vi "Demo_BjusticeData.vi"() -> ()   [LabVIEW 2021, in "RocketPlotDemo.lvlib"]
uses:
  Demo/RocketPlotDemo.lvlib
  TypeDefs/plot load data V2.ctl
  TypeDefs/plot properties V2.ctl
  TypeDefs/plot attributes V2.ctl
  TypeDefs/Plot scale axis properties.ctl
  TypeDefs/Plot general properties.ctl
  Classes/RocketPlotHandle/SubVIs/Init Options.ctl
  TypeDefs/TimeZone.ctl
  Classes/RocketPlotPanel/RocketPlotPanel.lvclass/RocketPlotPanel.ctl
  Classes/RocketPlotPanel/Read RocketPlotHandle.vi
  Classes/BjusticePlotHandle/BjusticePlotHandle.lvclass
  C:/Users/bjustice/Documents/GitHub/BluePlot/Source/Classes/RocketPlotHandle/RocketPlotHandle.lvclass
  Classes/RocketPlotPanel/RocketPlotPanel.lvclass
  C:/Program Files/National Instruments/LabVIEW 2021/vi.lib/IlluminatedG/IG OOPanel/OOPanel/Panel/Panel.lvclass
  Classes/RocketPlotHandle/Load PlotConfig.vi
  Classes/RocketPlotHandle/RocketPlotHandle.lvclass
  Classes/RocketPlotHandle/Get PlotConfig.vi
  RocketPlot.lvlib
  <userlib>/bjustice/Ring Buffer for Time Series Data Strict Accessor/Ring Buffer Strict Accessor.lvlib
  <vilib>/IlluminatedG/IG OOPanel/OOPanel/Manager/Manager.lvclass
  C:/Users/bjustice/Documents/GitHub/BluePlot/Source/Classes/BjusticePlotHandle/BjusticePlotHandle.lvclass
  C:/Users/bjustice/Documents/GitHub/BluePlot/Source/Classes/RocketPlotPanel/RocketPlotPanel.lvclass
panel:
  in  "load config":bool
  in  "get config":bool
  out "time to plot":dbl
  out "Subscribed names":i32(listbox)
  in  "Plot config":T1={"plots"=[], "X-axis"={"Name Label.Text"="", "Style"=0, "Tick Colors:Minor Tick Color"=0, "Tick Colors:Tick Color"=0, "Marker Colors:Text Color"=0, "Grid Colors:Major Color"=0, "Grid Colors:Minor Color"=0, "Mapping Mode"=0, "Flipped"=FALSE, "Name Label.Visible"=FALSE, "Name Label.Text Colors:Text Color"=0, "Scale Fit"=0, "Range:Maximum"=0.0, "Range:Minimum"=0.0, "Offset and Multiplier:Multiplier"=0.0, "Offset and Multiplier:Offset"=0.0, "Name Label.Font:Size"=0, "Marker.Font:Size"=0, "Uniform Marker Spacing?"=TRUE, "Format String"=""}, "Y-axes"=[], "General"={"Title"="", "Time to Plot"=1800.0, "Title.Visible"=FALSE, "Sidebar.Visible"=FALSE, "Plot Area:Colors:BG Color"=0, "X Scale.Plot Name"="", "X Scale.Use Plot Name"=FALSE}} {"General"."Time to Plot" format="%<%M:%S>t"}
  # "Documentation and user guide:"
  # "https://github.com/justiceb/BluePlot/blob/main/README.md"
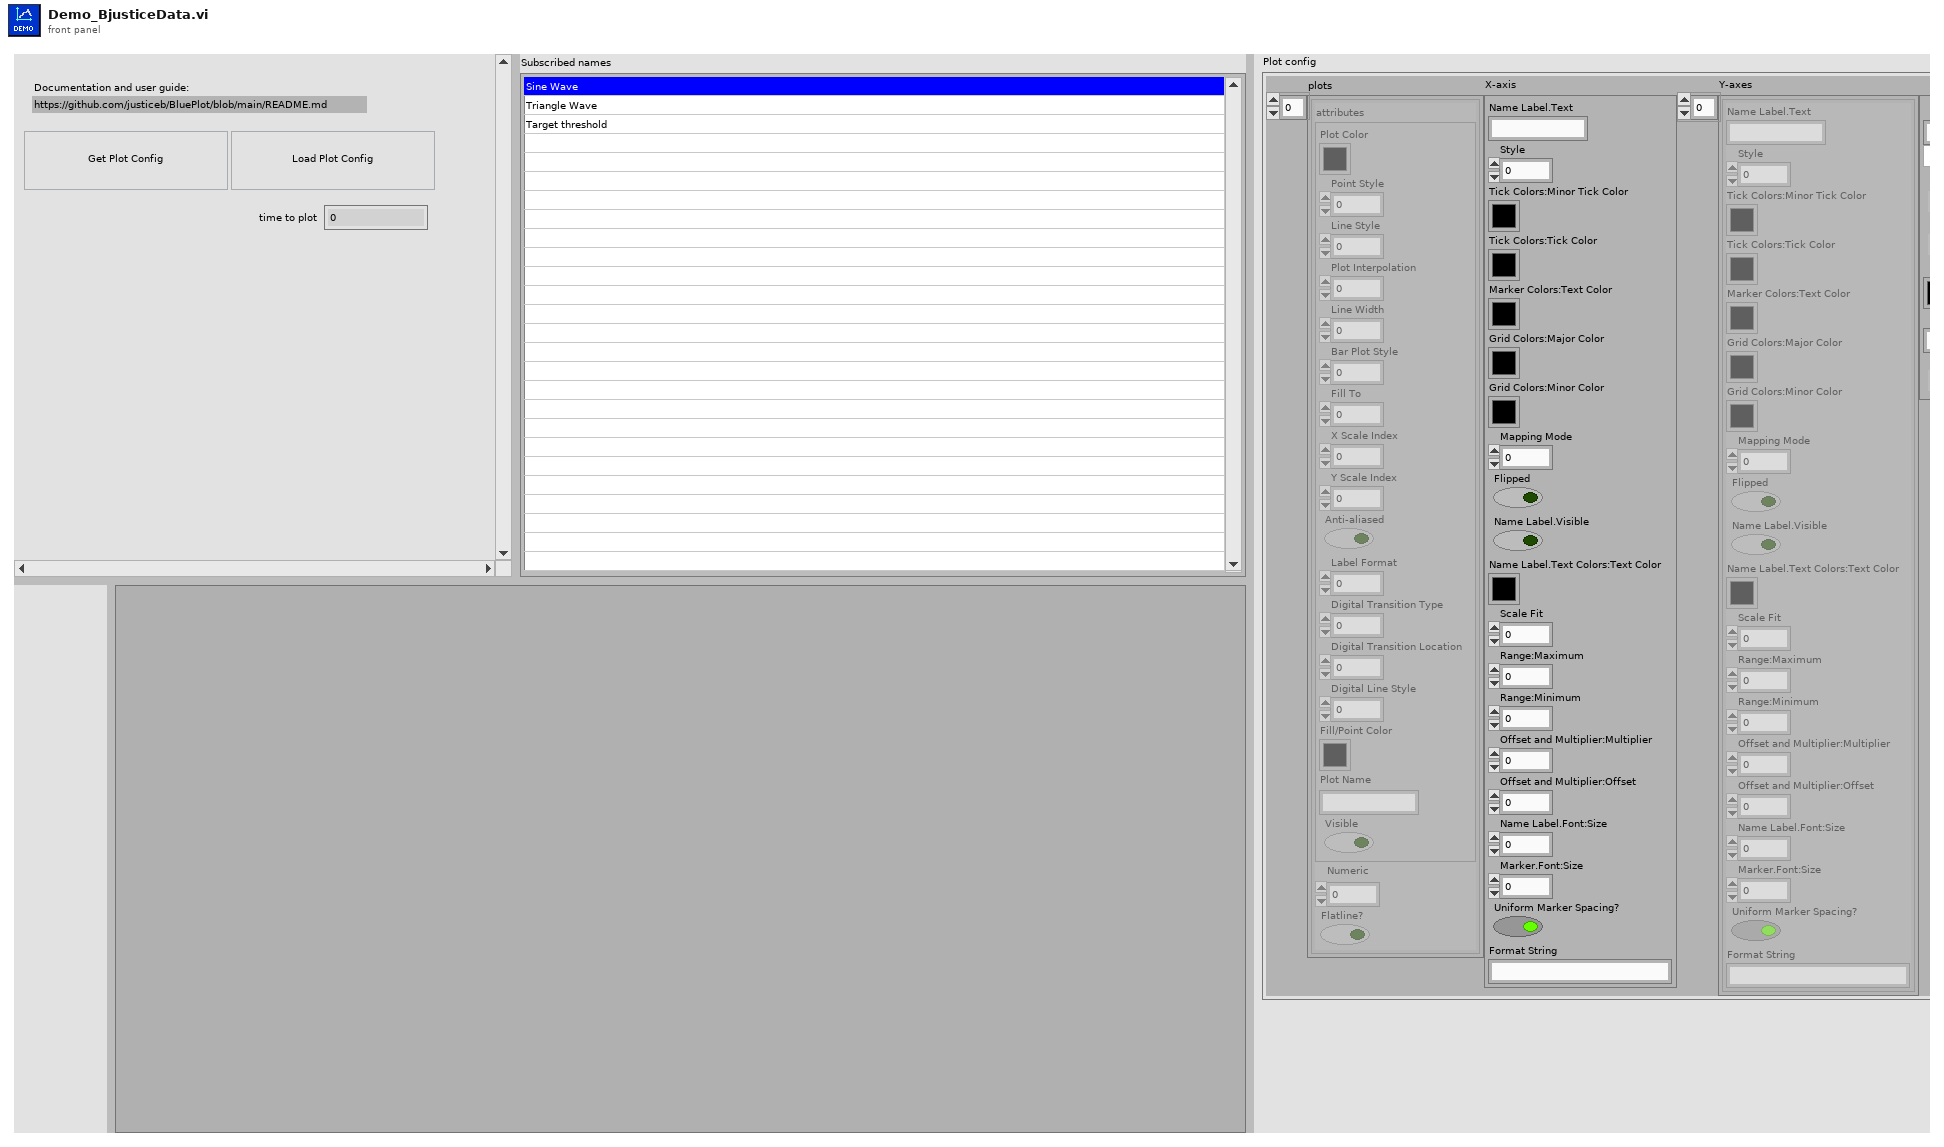
[diagram p1: front panel]
types:
  T1 = typedef "RocketPlot.lvlib/plot load data V2.ctl" = cluster{"plots":T2[], "X-axis":T4, "Y-axes":T4[], "General":T5}
  T2 = typedef "RocketPlot.lvlib/plot properties V2.ctl" = cluster{"attributes":T3, "Numeric":dbl, "Flatline?":bool}
  T3 = typedef "RocketPlot.lvlib/plot attributes V2.ctl" = cluster{"Plot Color":u32, "Point Style":u8, "Line Style":u8, "Plot Interpolation":u8, "Line Width":u8, "Bar Plot Style":u8, "Fill To":i16, "X Scale Index":u32, "Y Scale Index":u32, "Anti-aliased":bool, "Label Format":u8, "Digital Transition Type":u8, "Digital Transition Location":u8, "Digital Line Style":u8, "Fill/Point Color":u32, "Plot Name":string, "Visible":bool}
  T4 = typedef "RocketPlot.lvlib/Plot scale axis properties.ctl" = cluster{"Name Label.Text":string, "Style":u8, "Tick Colors:Minor Tick Color":u32, "Tick Colors:Tick Color":u32, "Marker Colors:Text Color":u32, "Grid Colors:Major Color":u32, "Grid Colors:Minor Color":u32, "Mapping Mode":u8, "Flipped":bool, "Name Label.Visible":bool, "Name Label.Text Colors:Text Color":u32, "Scale Fit":u8, "Range:Maximum":dbl, "Range:Minimum":dbl, "Offset and Multiplier:Multiplier":dbl, "Offset and Multiplier:Offset":dbl, "Name Label.Font:Size":u32, "Marker.Font:Size":u32, "Uniform Marker Spacing?":bool, "Format String":string}
  T5 = typedef "RocketPlot.lvlib/Plot general properties.ctl" = cluster{"Title":string, "Time to Plot":dbl, "Title.Visible":bool, "Sidebar.Visible":bool, "Plot Area:Colors:BG Color":u32, "X Scale.Plot Name":string, "X Scale.Use Plot Name":bool}
  T6 = typedef "RocketPlotHandle.lvclass/Init Options.ctl" = cluster{"UI visible?":bool, "Update rate (ms)":u32, "Sidebar.Visible":bool, "time to plot (init)":dbl, "time to plot (max)":dbl, "config file start path":path, "Title.Visible":bool, "Title":string, "TimeZone":T7}
  T7 = typedef "RocketPlot.lvlib/TimeZone.ctl" = enum16{"UTC", "Local"}
  T8 = typedef "Ring Buffer Strict Accessor.lvlib/RingBufferHandle.ctl" = cluster{"Ring buffer DVR":refnum<data-value>, "Data Type":T9, "Size(s)":i32[], "Endianess":T10, "Buffer Size (#timestamps) [init]":i32}
  T9 = typedef "Ring Buffer Strict Accessor.lvlib/DataType.ctl" = enum16{"uint8", "uint16", "uint32", "uint64", "int8", "int16", "int32", "int64", "float", "double", "extended"}
  T10 = typedef "Ring Buffer Strict Accessor.lvlib/Endianess.ctl" = enum16{"big-endian", "little-endian"}
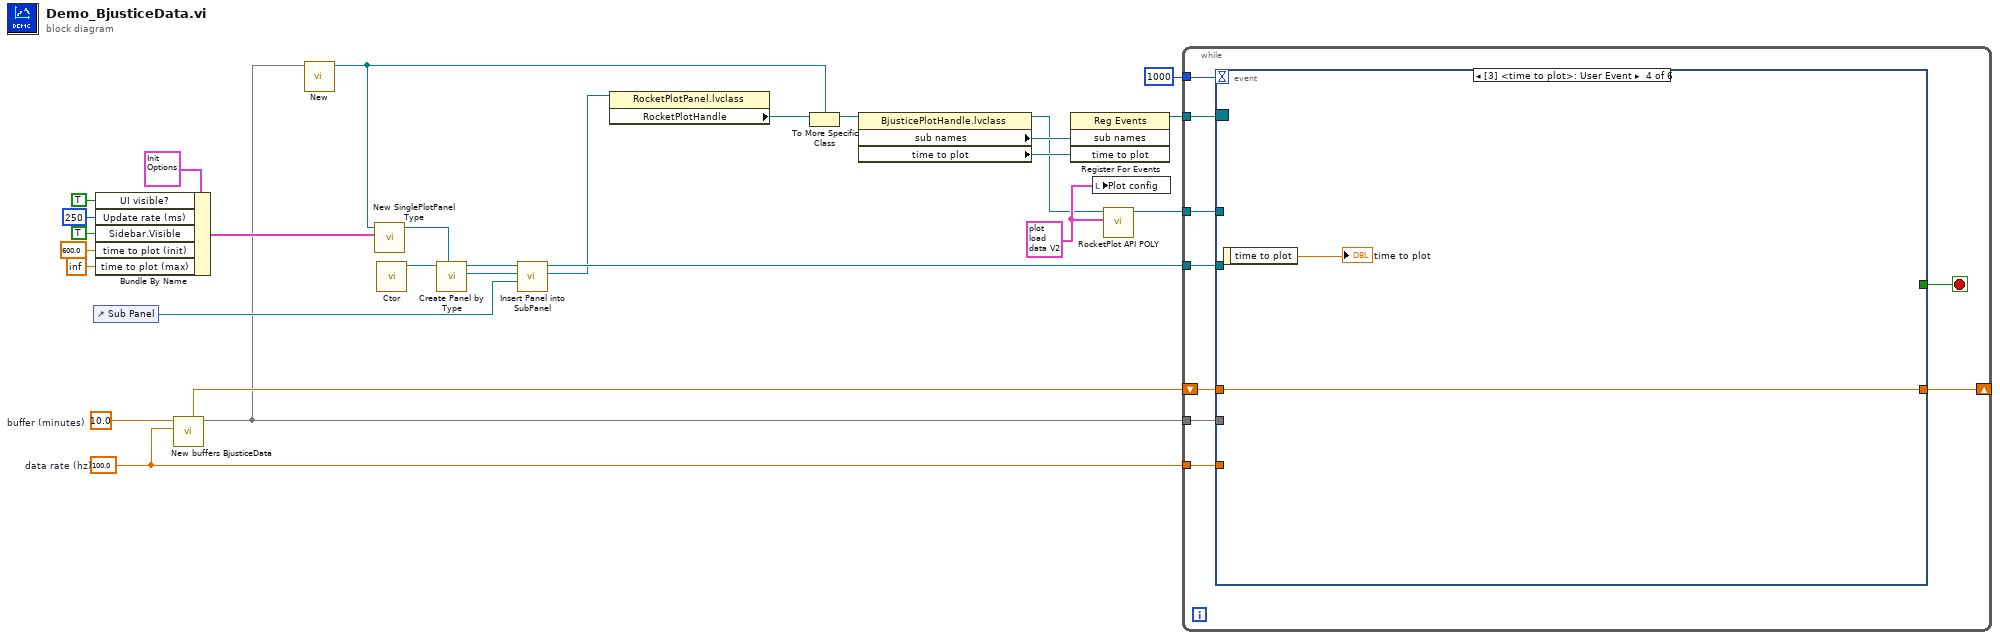
[diagram p0: block diagram]
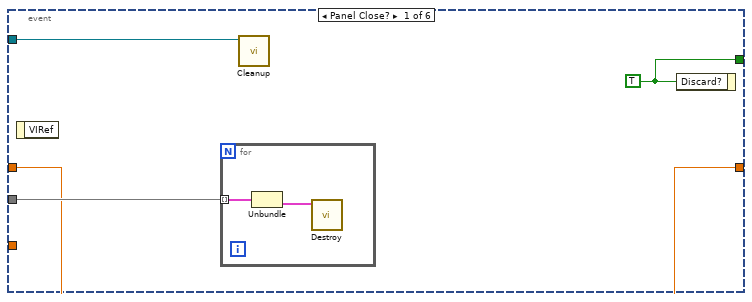
[diagram p2: hidden frame]
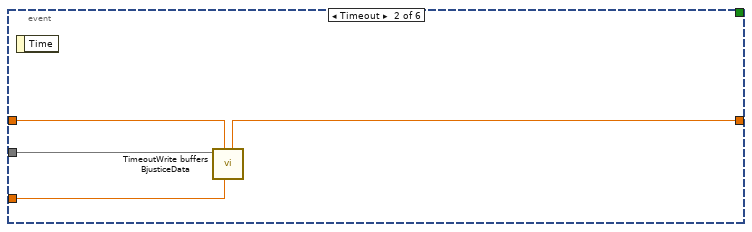
[diagram p3: hidden frame]
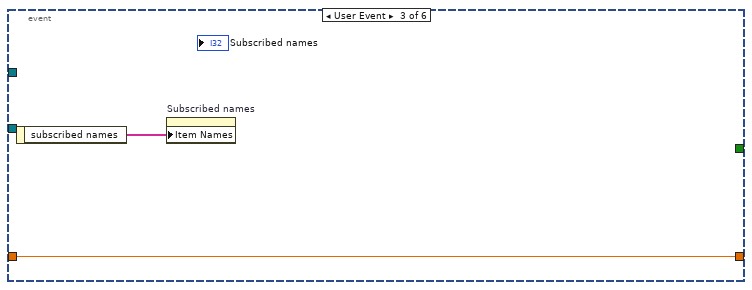
[diagram p4: hidden frame]
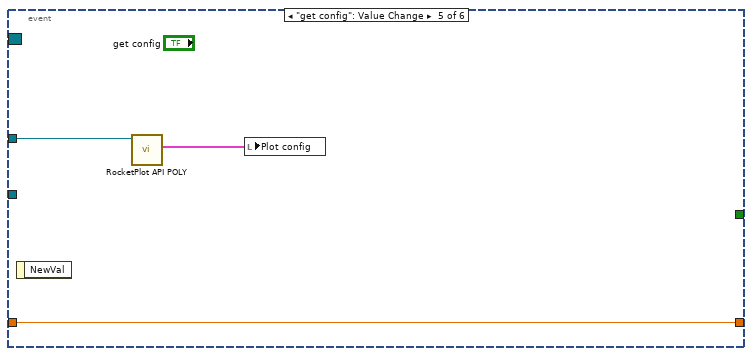
[diagram p5: hidden frame]
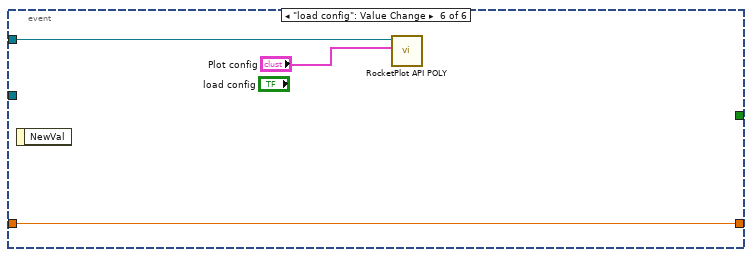
[diagram p6: hidden frame]
diagram:
  w20 = T1 {"plots"=[{"attributes"={"Plot Color"=16711680, "Point Style"=0, "Line Style"=0, "Plot Interpolation"=2, "Line Width"=0, "Bar Plot Style"=0, "Fill To"=-1, "X Scale Index"=0, "Y Scale Index"=0, "Anti-aliased"=FALSE, "Label Format"=3, "Digital Transition Type"=0, "Digital Transition Location"=2, "Digital Line Style"=1, "Fill/Point Color"=16711680, "Plot Name"="Sine Wave", "Visible"=TRUE}, "Numeric"=0.0, "Flatline?"=FALSE}, {"attributes"={"Plot Color"=4387583, "Point Style"=0, "Line Style"=0, "Plot Interpolation"=2, "Line Width"=0, "Bar Plot Style"=0, "Fill To"=-1, "X Scale Index"=0, "Y Scale Index"=1, "Anti-aliased"=FALSE, "Label Format"=3, "Digital Transition Type"=0, "Digital Transition Location"=2, "Digital Line Style"=1, "Fill/Point Color"=4387583, "Plot Name"="Triangle Wave", "Visible"=TRUE}, "Numeric"=0.0, "Flatline?"=FALSE}, {"attributes"={"Plot Color"=16722671, "Point Style"=0, "Line Style"=0, "Plot Interpolation"=2, "Line Width"=5, "Bar Plot Style"=0, "Fill To"=-1, "X Scale Index"=0, "Y Scale Index"=0, "Anti-aliased"=FALSE, "Label Format"=3, "Digital Transition Type"=0, "Digital Transition Location"=2, "Digital Line Style"=1, "Fill/Point Color"=16722671, "Plot Name"="Target threshold", "Visible"=TRUE}, "Numeric"=0.6, "Flatline?"=TRUE}, {"attributes"={"Plot Color"=16860, "Point Style"=0, "Line Style"=0, "Plot Interpolation"=2, "Line Width"=0, "Bar Plot Style"=0, "Fill To"=-1, "X Scale Index"=0, "Y Scale Index"=0, "Anti-aliased"=FALSE, "Label Format"=3, "Digital Transition Type"=0, "Digital Transition Location"=2, "Digital Line Style"=1, "Fill/Point Color"=16860, "Plot Name"="", "Visible"=TRUE}, "Numeric"=0.0, "Flatline?"=FALSE}], "X-axis"={"Name Label.Text"="Time (s)", "Style"=0, "Tick Colors:Minor Tick Color"=16777216, "Tick Colors:Tick Color"=3684408, "Marker Colors:Text Color"=16448250, "Grid Colors:Major Color"=3684408, "Grid Colors:Minor Color"=16777216, "Mapping Mode"=0, "Flipped"=FALSE, "Name Label.Visible"=TRUE, "Name Label.Text Colors:Text Color"=16448250, "Scale Fit"=2, "Range:Maximum"=3757348740.0, "Range:Minimum"=3757348080.0, "Offset and Multiplier:Multiplier"=1.0, "Offset and Multiplier:Offset"=0.0, "Name Label.Font:Size"=15, "Marker.Font:Size"=15, "Uniform Marker Spacing?"=TRUE, "Format String"="%<%H:%M:%S>T"}, "Y-axes"=[{"Name Label.Text"="Left Axis", "Style"=0, "Tick Colors:Minor Tick Color"=16777216, "Tick Colors:Tick Color"=3684408, "Marker Colors:Text Color"=16448250, "Grid Colors:Major Color"=3684408, "Grid Colors:Minor Color"=16777216, "Mapping Mode"=0, "Flipped"=FALSE, "Name Label.Visible"=FALSE, "Name Label.Text Colors:Text Color"=16448250, "Scale Fit"=2, "Range:Maximum"=1.0, "Range:Minimum"=-1.0, "Offset and Multiplier:Multiplier"=1.0, "Offset and Multiplier:Offset"=0.0, "Name Label.Font:Size"=15, "Marker.Font:Size"=15, "Uniform Marker Spacing?"=TRUE, "Format String"="%#_g"}, {"Name Label.Text"="Right Axis", "Style"=0, "Tick Colors:Minor Tick Color"=16777216, "Tick Colors:Tick Color"=3684408, "Marker Colors:Text Color"=16448250, "Grid Colors:Major Color"=3684408, "Grid Colors:Minor Color"=16777216, "Mapping Mode"=0, "Flipped"=FALSE, "Name Label.Visible"=FALSE, "Name Label.Text Colors:Text Color"=16448250, "Scale Fit"=0, "Range:Maximum"=1.0, "Range:Minimum"=-2.0, "Offset and Multiplier:Multiplier"=1.0, "Offset and Multiplier:Offset"=0.0, "Name Label.Font:Size"=15, "Marker.Font:Size"=15, "Uniform Marker Spacing?"=TRUE, "Format String"="%#_g"}], "General"={"Title"="Title", "Time to Plot"=600.0, "Title.Visible"=TRUE, "Sidebar.Visible"=TRUE, "Plot Area:Colors:BG Color"=0, "X Scale.Plot Name"="", "X Scale.Use Plot Name"=FALSE}} ("Plot config")
  w17 = 100.0  # data rate (hz)
  w19 = 10.0  # buffer (minutes)
  n1 = control-ref of="Sub Panel"() -> (w11:refnum<vi>)
  n2 = Bundle By Name(cluster=T6 {"UI visible?"=TRUE, "Update rate (ms)"=250, "Sidebar.Visible"=TRUE, "time to plot (init)"=600.0, "time to plot (max)"=inf, "config file start path"=path "", "Title.Visible"=TRUE, "Title"="Title", "TimeZone"=enum."Local"} ("Init options"), "UI visible?"=TRUE, "Update rate (ms)"=u32 250, "Sidebar.Visible"=TRUE ("visible sidebar?"), "time to plot (init)"=600.0, "time to plot (max)"=inf) -> (w14:T6)
  n3 = call "New buffers BjusticeData.vi"("data rate (hz)"=w17, "buffer (minutes)"=w19) -> ("Map"=w7:map{string, T8}, "last timestamp"=w16:dbl)  [unwired: 8 in]
  n4 = call "New.vi"("ChannelMap"=w7) -> ("StokePlotHandle out"=w5:refnum<class "BjusticePlotHandle.lvclass">)  [unwired: 9 in, 1 out]
  n5 = call "New SinglePlotPanel Type.vi"("Init options"=w14, "BluePlotHandle"=w5) -> ("SinglePlotPanel out"=w13:refnum<class "RocketPlotPanel.lvclass">)  [unwired: 8 in, 1 out]
  n6 = call <vilib>:"Ctor.vi"() -> ("Manager out"=w15:refnum<class "Manager.lvclass">)  [unwired: 10 in, 1 out]
  n7 = call <vilib>:"Create Panel by Type.vi"("Panel Type"=w13, "Manager in"=w15) -> ("Panel"=w10:refnum<class "RocketPlotPanel.lvclass">, "Manager out"=w12:refnum<class "Manager.lvclass">)  [unwired: 7 in, 1 out]
  n8 = call <vilib>:"Insert Panel into SubPanel.vi"("SubPanel"=w11, "Panel In"=w10, "Manager in"=w12) -> ("Panel"=w8:refnum<class "RocketPlotPanel.lvclass">, "Manager out"=w9:refnum<class "Manager.lvclass">)  [unwired: 6 in, 1 out]
  n9 = property class="RocketPlotPanel.lvclass"(reference=w8) -> ("RocketPlotHandle"=w6:refnum<class "RocketPlotHandle.lvclass">)  [unwired: 1 in, 2 out]
  n10 = To More Specific Class(target class=w5, reference=w6) -> (specific class reference=w4:refnum<class "BjusticePlotHandle.lvclass">)  [unwired: 1 in, 1 out]
  n11 = property class="BjusticePlotHandle.lvclass"(reference=w4) -> (reference out=w1:refnum<class "BjusticePlotHandle.lvclass">, "sub names"=w3:refnum<user-event>, "time to plot"=w2:refnum<user-event>)  [unwired: 1 in, 1 out]
  n12 = register-events(w3, w2) -> (reference out=w28:refnum<event-registration>)  [unwired: 2 in, 1 out]
  n13 = local write "Plot config"(w20) -> ()
  n14 = call-poly "RocketPlot API POLY.vi"("Plot config"=w20, "BluePlotHandle in"=w1) -> ("BluePlotHandle out"=w21:refnum<class "BjusticePlotHandle.lvclass">)  [unwired: 8 in, 1 out]
  n15 = while {
    tunnel: w21 -> [w37]
    tunnel: w28 -> [w35]
    tunnel: w7 -> [w34]
    tunnel: 1000 ("period (ms)") -> [w33]
    shift-right: [w31] -> _
    shift-left: w16 -> [w32]
    tunnel: w17 -> [w30]
    tunnel: w9 -> [w29]
    stop <- w36 stop-if-true
    n16 = event shown="[3] <time to plot>: User Event" {
      selector: w35 -> [_ _ _ _ _ _]
      dyn-events: _ -> [_ _ _ _ _ _]
      timeout: w33 -> [_ _ _ _ _ _]
      tunnel: w37 -> [_ _ _ _ w54 w57]
      tunnel: [w40 _ _ _ _ _] -> w36
      tunnel: w34 -> [w41 w47 _ _ _ _]
      tunnel: w32 -> [w39 w46 w48 w50 w52 w55]
      tunnel: [w39 w45 w48 w50 w52 w55] -> w31
      tunnel: w30 -> [_ w44 _ _ _ _]
      tunnel: w29 -> [w38 _ _ _ _ _]
      event Panel Close? {
        w40 = TRUE ("Discard?")
        n17 = event-data() -> ()  [unwired: 1 in, 1 out]
        n18 = for {
          tunnel: w41 -> [w43] mode=indexing
          n19 = Unbundle(w43) -> ("Ring Buffer"=w42:T8)  [unwired: 1 out]
          n20 = call <userlib>:"Destroy.vi"("Ring Buffer"=w42) -> ()  [unwired: 10 in, 1 out]
        }
        n21 = call <vilib>:"Cleanup.vi"("Manager in"=w38) -> ()  [unwired: 8 in, 3 out]
        n22 = event-data("Discard?"=w40) -> ()  [unwired: 1 in, 1 out]
      }
      event Timeout {
        n23 = event-data() -> ()  [unwired: 1 in, 1 out]
        n24 = call "TimeoutWrite buffers BjusticeData.vi"("data rate (hz)"=w44, "previous timestamp"=w46, "Map"=w47) -> ("current timestamp"=w45:dbl)  [unwired: 8 in]
      }
      event User Event {
        n25 = event-data() -> ("subscribed names"=w49:string[])  [unwired: 1 in]
        n26 = property on="Subscribed names" class="LstBox (strict)"("Item Names"=w49) -> ()  [unwired: 2 in, 2 out]
      }
      event User Event {
        n27 = event-data() -> ("time to plot"=→"time to plot":dbl)  [unwired: 1 in]
      }
      event "get config": Value Change {
        n28 = event-data() -> ()  [unwired: 1 in, 1 out]
        n29 = call-poly "RocketPlot API POLY.vi"("BluePlotHandle in"=w54) -> ("Plot config"=w53:T1)  [unwired: 8 in, 2 out]
        n30 = local write "Plot config"(w53) -> ()
      }
      event "load config": Value Change {
        n31 = event-data() -> ()  [unwired: 1 in, 1 out]
        n32 = call-poly "RocketPlot API POLY.vi"("Plot config"="Plot config", "BluePlotHandle in"=w57) -> ()  [unwired: 8 in, 2 out]
      }
    }
  }
